vi "Native_GetTunnelTerminals_v2.vi"() -> ()   [LabVIEW 2024]
panel:
  out "error out":errorcluster caption="错误输出"
  out "outside_id":u32
  in  "outside_id type":u32
  out "inside_ids":u32[](array[numeric])
  in  "inside_ids type":u32
  in  "tunnel_id":u32
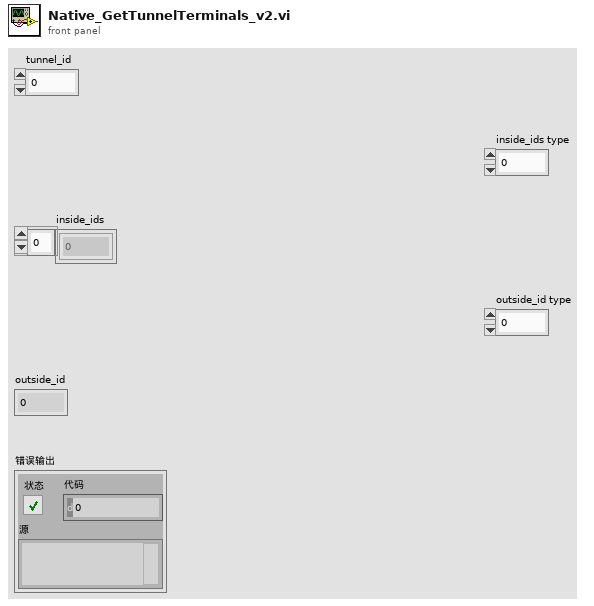
[diagram p1: front panel]
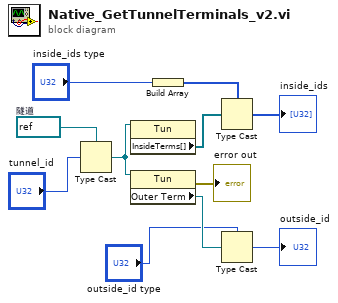
[diagram p0: block diagram]
diagram:
  w10 = refnum<vi> refnum  # 隧道
  n1 = Type Cast ("强制类型转换")(type=w10, x="tunnel_id") -> (*(type *) &x=w9:refnum<vi>)
  n2 = property on="属性节点" class="Tun"(reference=w9) -> ("InsideTerms[]"=w8:refnum<vi>[])  [unwired: 1 in, 2 out]
  n3 = property on="属性节点" class="Tun"(reference=w9) -> (error out=→"error out":errorcluster, "Outer Term"=w4:refnum<vi>)  [unwired: 1 in, 1 out]
  n4 = Build Array ("创建数组")("inside_ids type") -> (w6:u32[])
  n5 = Type Cast ("强制类型转换")(type=w6, x=w8) -> (*(type *) &x=→"inside_ids":u32[])
  n6 = Type Cast ("强制类型转换")(type="outside_id type", x=w4) -> (*(type *) &x=→"outside_id":u32)
